vi "Configure Parallel Execution.vi"(8 "error in (no error)":errorcluster, 9 "Persist?":bool, 10 "Enable Parallel Execution?":bool, 11 "Execution UI In":refnum<class "Execution UI.lvclass">) -> (0 "error out":errorcluster, 3 "Execution UI Out":refnum<class "Execution UI.lvclass">)   [LabVIEW 2020, in "Execution UI.lvclass"]
uses:
  Execution UI.lvclass
  Execution UI.lvclass/Execution UI.ctl
  Configuration Manager/UI Configuration Manager.lvclass
  Framework/Single Thread Test Runner/Single Thread Test Runner.lvclass
  Framework/Parallel Test Runner/Parallel Test Runner.lvclass
  Framework/Test Runner/Test Runner.lvclass
  C:/git/astemes-lunit/source/Framework/Single Thread Test Runner/Single Thread Test Runner.lvclass
  C:/git/astemes-lunit/source/Framework/Test Runner/Test Runner.lvclass
  C:/git/astemes-lunit/source/Framework/Parallel Test Runner/Parallel Test Runner.lvclass
  C:/git/astemes-lunit/source/User Interface/Execution UI/Execution UI.lvclass
  C:/git/astemes-lunit/source/Framework/Result Observer/Result Observer.lvclass
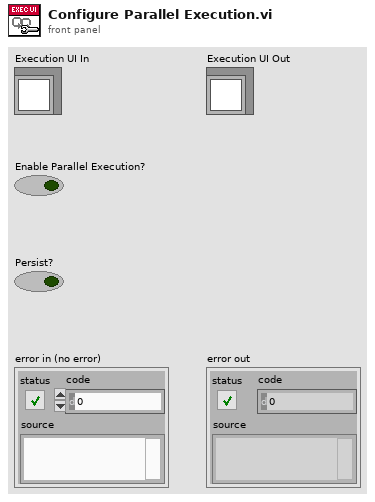
[diagram p1: front panel]
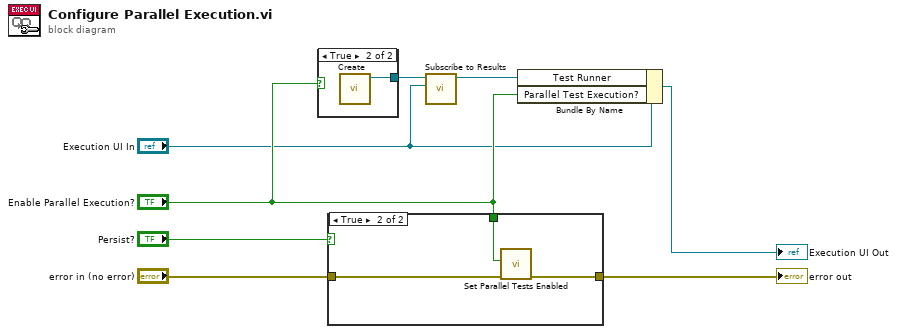
[diagram p0: block diagram]
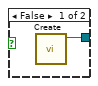
[diagram p3: hidden frame]
diagram:
  n1 = case shown="True" "Enable Parallel Execution?" {
    tunnel: [w9 w10] -> w5
    frame False {
      n2 = call "Create.vi"() -> ("Single Thread Test Runner out"=w9:refnum<class "Single Thread Test Runner.lvclass">)  [unwired: 10 in, 1 out]
    }
    frame True {
      n3 = call "Create.vi"() -> ("Parallell Test Runner out"=w10:refnum<class "Parallel Test Runner.lvclass">)  [unwired: 10 in, 1 out]
    }
  }
  n4 = case shown="True" "Persist?" {
    tunnel: "Enable Parallel Execution?" -> [_ w14]
    tunnel: [w11 w12] -> w4
    tunnel: "error in (no error)" -> [w11 w13]
    frame False {
    }
    frame True {
      n5 = call "Set Parallel Tests Enabled.vi"("error in (no error)"=w13, "Parallel tests enabled?"=w14) -> ("error out"=w12:errorcluster)  [unwired: 9 in]
    }
  }
  "error out" <- w4
  n6 = call-dynamic "Subscribe to Results.vi"("Result Observer"="Execution UI In", "Test Runner In"=w5) -> ("Test Runner Out"=w7:refnum<class "Test Runner.lvclass">)  [unwired: 8 in, 1 out]
  n7 = Bundle By Name(cluster="Execution UI In", "Test Runner"=w7, "Parallel Test Execution?"="Enable Parallel Execution?") -> (→"Execution UI Out":refnum<class "Execution UI.lvclass">)
